vi "Create Manager.Text.vi"(4 "write delay (ms)":i32, 5 "ConfigManager.Text":refnum<class "ConfigManager.Text.lvclass">, 6 "read-only?":bool, 8 "error in (no error)":errorcluster, 9 "Create if Non Existent? (T)":bool=TRUE, 11 "filepath":path) -> (0 "error out":errorcluster, 2 "CfgManager.Text Public Events":T1, 3 "ConfigManager.Text out":refnum<class "ConfigManager.Text.lvclass">)   [LabVIEW 2013, in "CfgManager.Text.lvlib" / "ConfigManager.Text.lvclass"]
uses:
  ConfigManager.Text.lvclass
  PublicEvents -- Cluster.ctl
  payload -- cluster.ctl
  Response - cluster.ctl
  Manager/ConfigManager.lvclass/ConfigManager.ctl
  ConfigManager.Text.lvclass/ConfigManager.Text.ctl
  Manager/ConfigManager.lvclass
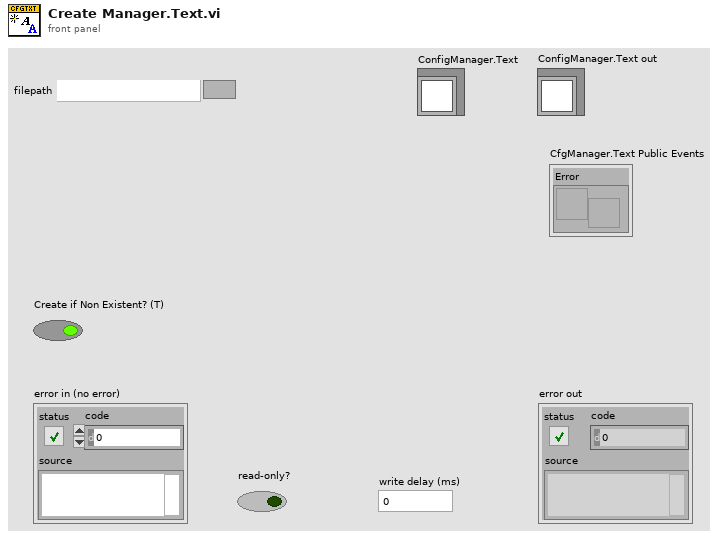
[diagram p1: front panel]
types:
  T1 = typedef "CfgManager.Text.lvlib/ConfigManager.Text.lvclass/PublicEvents -- Cluster.ctl" = cluster{"Error":refnum<user-event>}
  T2 = typedef "CfgManager.Text.lvlib/ConfigManager.Text.lvclass/payload -- cluster.ctl" = cluster{"command":string, "args":variant, "query":refnum<notifier>, "ack":refnum<notifier>}
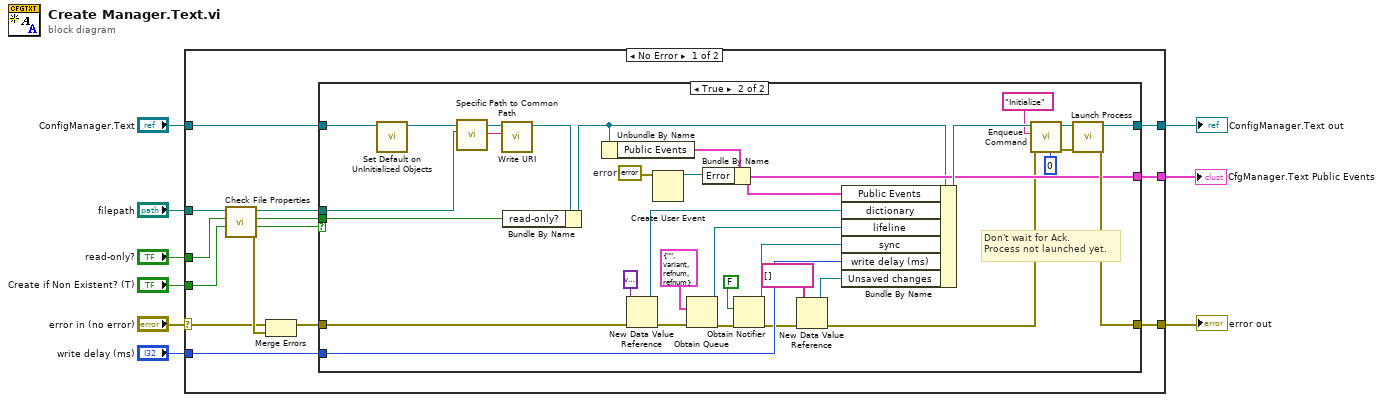
[diagram p0: block diagram]
diagram:
  n1 = case shown="No Error" "error in (no error)" {
    selector: "error in (no error)" -> [w14 w58]
    tunnel: "ConfigManager.Text" -> [w22 w59]
    tunnel: [w21 w59] -> w3
    tunnel: "filepath" -> [w20 _]
    tunnel: [w23 w58] -> w6
    tunnel: "read-only?" -> [w18 _]
    tunnel: [w12 _] -> w4
    tunnel: "write delay (ms)" -> [w11 _]
    tunnel: "Create if Non Existent? (T)" -> [w10 _]
    frame No Error {
      n2 = call "Check File Properties.vi"("Create if Non Existent?"=w10, "Read-Only?"=w18, "filepath"=w20) -> ("error out"=w15:errorcluster, "File exists"=w16:bool, "Read-Only"=w17:bool, "filepath dup"=w19:path)  [unwired: 4 in, 1 out]
      n3 = Merge Errors(w14, w15) -> (w13:errorcluster)
      n4 = case shown="True" w16 {
        tunnel: [w24 w54] -> w23
        tunnel: w22 -> [w25 w42]
        tunnel: [w25 w37] -> w21
        tunnel: w13 -> [w24 w44]
        tunnel: w19 -> [_ w32]
        tunnel: w17 -> [_ w33]
        tunnel: [_ w38] -> w12
        tunnel: w11 -> [_ w30]
        frame False {
        }
        frame True {
          w40 = errorcluster {"status"=FALSE, "code"=0, "source"=""}  # error
          # "Don't wait for Ack.\nProcess not launched yet."
          n5 = call "Set Default on UnInitialized Objects.vi"("ConfigManager.Text in"=w42) -> ("ConfigManager.Text out"=w36:refnum<class "ConfigManager.Text.lvclass">)  [unwired: 10 in]
          n6 = call "Specific Path to Common Path.vi"("specific path"=w32) -> ("common path"=w31:string)  [unwired: 10 in]
          n7 = call "Write URI.vi"("URI"=w31, "ConfigManager in"=w36) -> ("ConfigManager out"=w35:refnum<class "ConfigManager.Text.lvclass">)  [unwired: 9 in]
          n8 = Bundle By Name(cluster=w35, "read-only?"=w33) -> (w34:refnum<class "ConfigManager.Text.lvclass">)
          n9 = Unbundle By Name(w34) -> ("Public Events"=w39:T1)
          n10 = New Data Value Reference(data value=variant ("Variant"), error in=w44) -> (data value reference=w56:refnum<data-value>, error out=w43:errorcluster)
          n11 = Create User Event(user event datatype=w40) -> (user event=w41:refnum<user-event>)  [unwired: 1 in, 1 out]
          n12 = Obtain Queue(element data type=T2 {"command"="", "args"=variant, "query"=refnum, "ack"=refnum} ("payload"), error in (no error)=w43) -> (queue out=w47:refnum<queue>, error out=w45:errorcluster)  [unwired: 3 in, 1 out]
          n13 = Bundle By Name(cluster=w39, "Error"=w41) -> (w38:T1)
          n14 = Obtain Notifier(notification data type=FALSE, error in (no error)=w45) -> (notifier out=w46:refnum<notifier>, error out=w29:errorcluster)  [unwired: 2 in, 1 out]
          n15 = New Data Value Reference(data value=string[] [], error in=w29) -> (data value reference=w27:refnum<data-value>, error out=w28:errorcluster)
          n16 = Bundle By Name(cluster=w34, "Public Events"=w38, "dictionary"=w56, "lifeline"=w47, "sync"=w46, "write delay (ms)"=w30, "Unsaved changes"=w27) -> (w52:refnum<class "ConfigManager.Text.lvclass">)
          n17 = call "Enqueue Command.vi"("ack timeout (0 ms: no ack)"=0 ("ack timeout (ms)"), "error in (no error)"=w28, "command"="Initialize", "ConfigManager.Text in"=w52) -> ("error out"=w48:errorcluster, "ConfigManager.Text out"=w51:refnum<class "ConfigManager.Text.lvclass">)  [unwired: 5 in, 1 out]
          n18 = call-dynamic "Launch Process.vi"("error in (no error)"=w48, "ConfigManager.Text in"=w51) -> ("error out"=w54:errorcluster, "ConfigManager.Text out"=w37:refnum<class "ConfigManager.Text.lvclass">)  [unwired: 7 in, 1 out]
        }
      }
    }
    frame Error {
    }
  }
  "ConfigManager.Text out" <- w3
  "error out" <- w6
  "CfgManager.Text Public Events" <- w4
